vi "Create Type Definitions.vi"(8 "error in":errorcluster, 11 "IRunner in":refnum<class "IRunner.lvclass">) -> (0 "error out":errorcluster, 3 "IRunner out":refnum<class "IRunner.lvclass">)   [LabVIEW 2026, in "IRunner.lvlib" / "IRunner.lvclass"]
doc: "Create type definitions."
uses:
  IRunner.lvclass
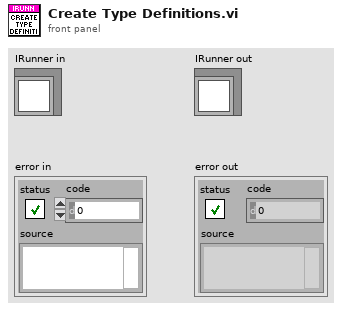
[diagram p1: front panel]
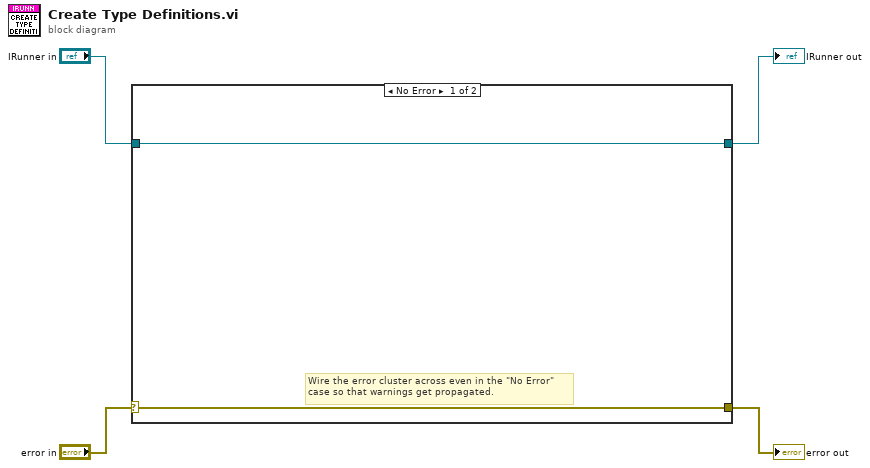
[diagram p0: block diagram]
diagram:
  n1 = case shown="No Error" "error in" {
    selector: "error in" -> [w6 w8]
    tunnel: [w6 w8] -> w3
    tunnel: [w5 w7] -> w1
    tunnel: "IRunner in" -> [w5 w7]
    frame No Error {
      # "Wire the error cluster across even in the \"No Error\"\ncase so that warnings get propagated."
    }
    frame Error {
    }
  }
  "error out" <- w3
  "IRunner out" <- w1
